vi "SPI Open.vi"(8 "error in (no error)":errorcluster, 9 "Mode":T1, 10 "Speed":i32=4000000, 11 "SPI Device":T2) -> (0 "error out":errorcluster, 3 "SPI Device out":T2)   [LabVIEW 2020, in "wiringPi.lvlib"]
doc: "<b>_______________________________________________________________</b>\n** Author: Juan José Villacorta\n** LabVIEW wrapper for C library <b> wiringPi </b>,\n** https://github.com/WiringPi/WiringPi\n<b>_______________________________________________________________</b>\n/*\n * Opens and configures a SPI Device\n**********************************************************************************\n*/"
uses:
  wiringPi.lvlib
  Type Defs/SPI Dev.ctl
  Type Defs/SPI Channel.ctl
  Type Defs/SPI Device.ctl
  Type Defs/SPI Mode.ctl
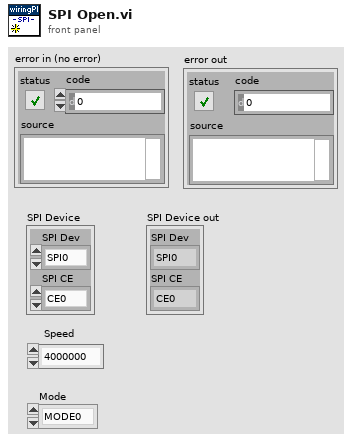
[diagram p1: front panel]
types:
  T1 = typedef "wiringPi.lvlib/SPI Mode.ctl" = enum32{"MODE0", "MODE1", "MODE2", "MODE3"}
  T2 = typedef "wiringPi.lvlib/SPI Device.ctl" = cluster{"SPI Dev":T3, "SPI CE":T4}
  T3 = typedef "wiringPi.lvlib/SPI Dev.ctl" = enum32{"SPI0", "SPI1"}
  T4 = typedef "wiringPi.lvlib/SPI Channel.ctl" = enum32{"CE0", "CE1", "CE2"}
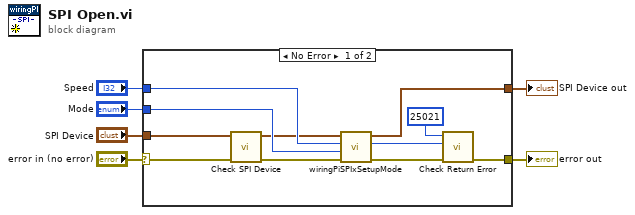
[diagram p0: block diagram]
diagram:
  n1 = case shown="No Error" "error in (no error)" {
    selector: "error in (no error)" -> [w15 w19]
    tunnel: [w9 w19] -> w5
    tunnel: "SPI Device" -> [w13 w18]
    tunnel: "Speed" -> [w17 _]
    tunnel: "Mode" -> [w16 _]
    tunnel: [w11 w18] -> w1
    frame No Error {
      n2 = call "Check SPI Device.vi"("error in (no error)"=w15, "SPI Device"=w13) -> ("error out"=w14:errorcluster, "SPI Device out"=w12:T2)  [unwired: 8 in]
      n3 = call "wiringPiSPIxSetupMode.vi"("error in (no error)"=w14, "Mode"=w16, "Speed"=w17, "SPI Device"=w12) -> ("error out"=w10:errorcluster, "return"=w8:i32, "SPI Device out"=w11:T2)  [unwired: 5 in]
      n4 = call "Check Return Error.vi"("error in (no error)"=w10, "Return code"=w8, "Error number"=25021) -> ("error out"=w9:errorcluster)  [unwired: 8 in]
    }
    frame Error {
    }
  }
  "error out" <- w5
  "SPI Device out" <- w1
